vi "Save Profi map Power.vi"(7 "Write":bool, 8 "error in":errorcluster, 10 "configuration file path":path, 11 "Power Meters":cluster{"Select Item 3":T2, "Combo Box 2":T4}[](array[cluster])) -> (0 "error out":errorcluster, 3 "Array":cluster{"Sensor":T1, "Profi":T2}[](array[cluster]))   [LabVIEW 2025]
uses:
  <vilib>/Utility/config.llb/NI_LVConfig.lvlib
  controls/Tempratures.ctl
  controls/Profi address.ctl
  <vilib>/Utility/config.llb/Read Key (String).vi
  <vilib>/Utility/config.llb/Write Key (String).vi
  controls/Power Meters.ctl
panel:
  in  "Pressure":T3(array[cluster])
  in  "Tempratures":cluster{"Sensor":T1, "Profi":T2}[][](array[cluster])
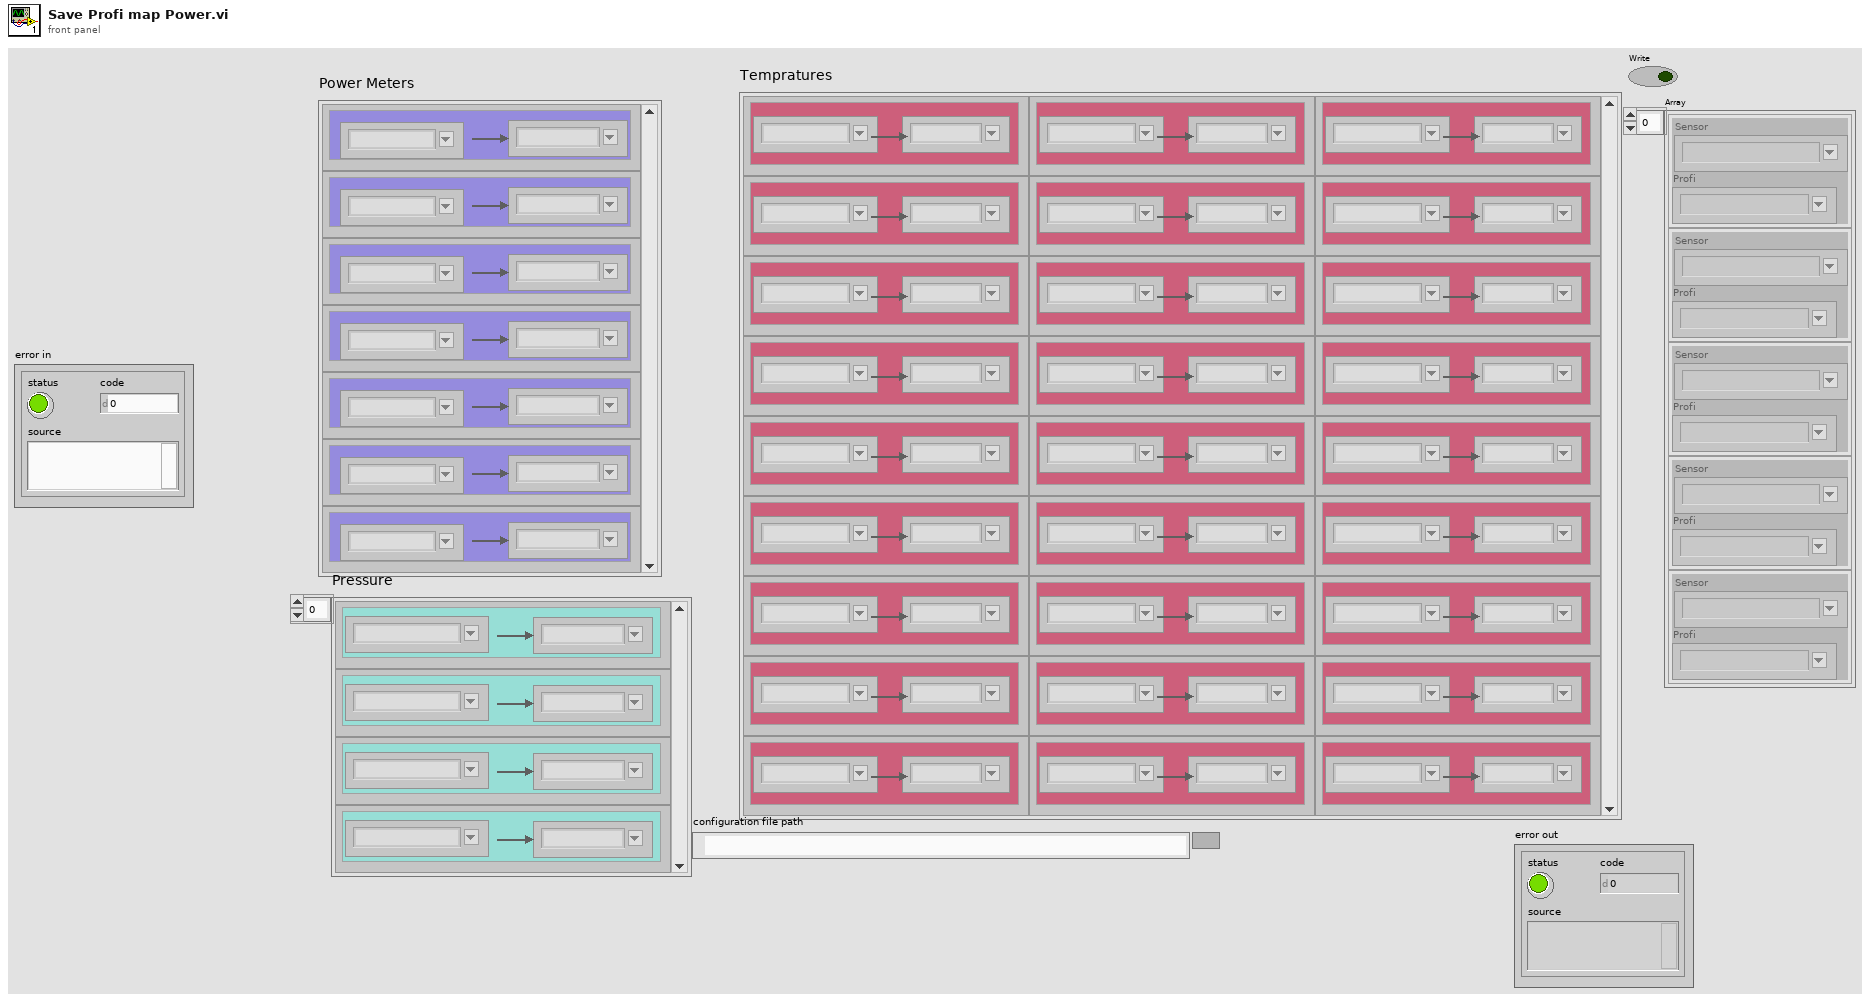
[diagram p1: front panel]
types:
  T1 = typedef "Tempratures.ctl" = string
  T2 = typedef "Profi address.ctl" = string
  T3 = cluster{"Select Item 3":T2, "Combo Box 2":string}[]
  T4 = typedef "Power Meters.ctl" = string
  T5 = typedef "NI_LVConfig.lvlib/Config Data RefNum.ctl" = refnum<k1>
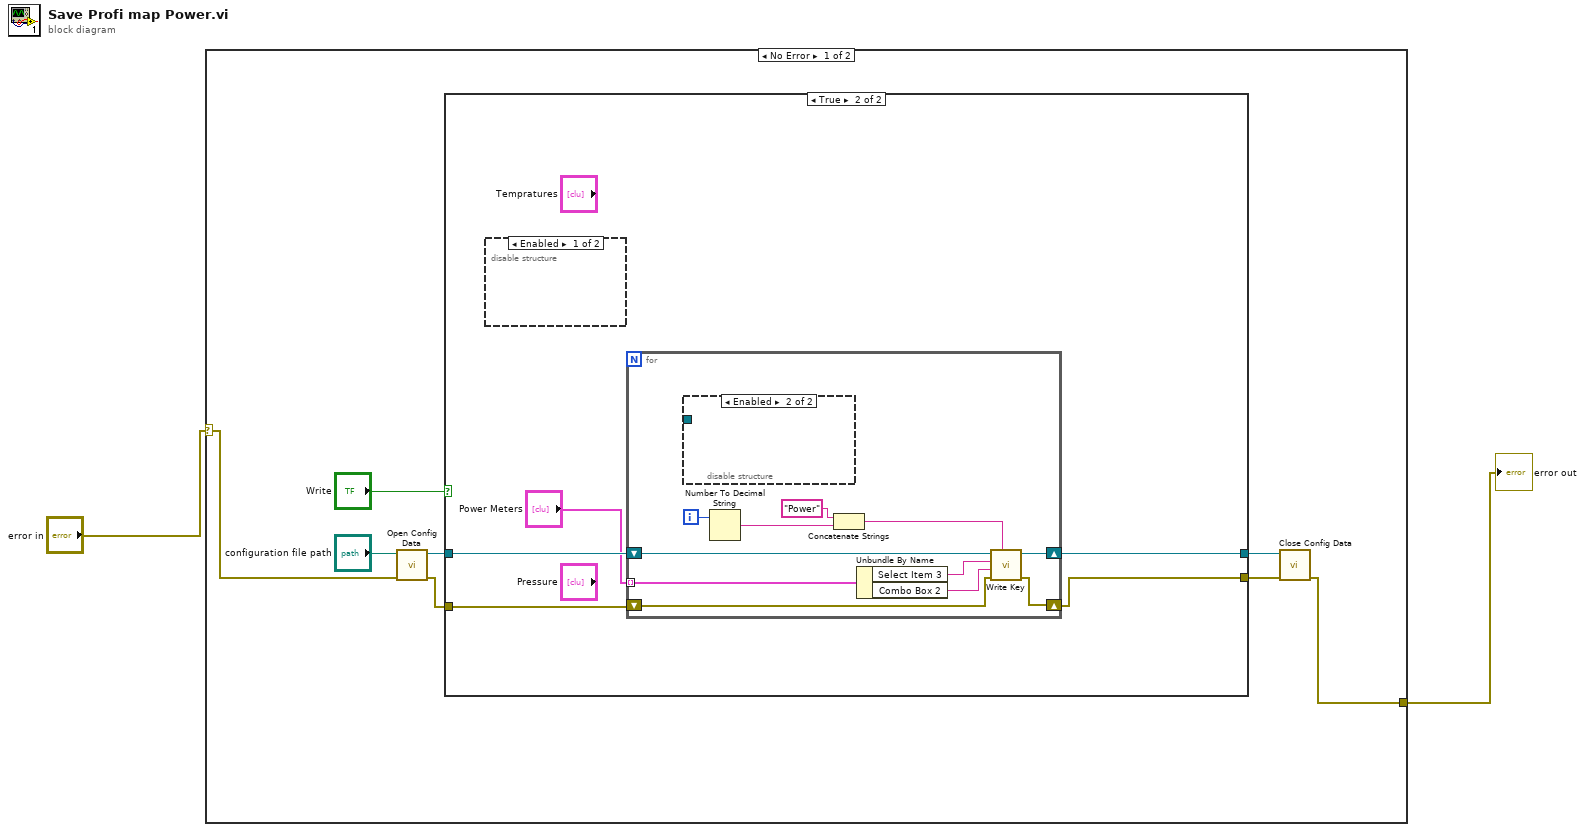
[diagram p0: block diagram]
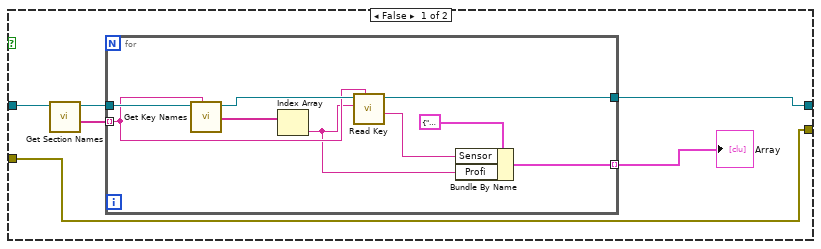
[diagram p2: hidden frame]
diagram:
  n1 = case shown="No Error" "error in" {
    selector: "error in" -> [w6 w43]
    tunnel: [w3 w43] -> w1
    frame No Error {
      n2 = call <vilib>:"Open Config Data.vi"("error in (no error)"=w6, "configuration file path"="configuration file path") -> ("error out"=w5:errorcluster, "refnum"=w10:T5)  [unwired: 7 in, 1 out]
      n3 = case shown="True" "Write" {
        tunnel: w10 -> [w15 w30]
        tunnel: [w16 w29] -> w7
        tunnel: w5 -> [w12 w27]
        tunnel: [w12 w26] -> w4
        frame False {
          n4 = call <vilib>:"Get Section Names.vi"("refnum"=w15) -> ("section names"=w14:string[], "refnum out"=w13:T5)  [unwired: 8 in, 1 out]
          n5 = for {
            tunnel: [w25] -> w16
            tunnel: w14 -> [w20] mode=indexing
            tunnel: w13 -> [w23]
            tunnel: [w22] -> w11 mode=indexing
            n6 = call <vilib>:"Get Key Names.vi"("section"=w20, "refnum"=w23) -> ("key names"=w19:string[], "refnum out"=w24:T5)  [unwired: 6 in, 2 out]
            n7 = Index Array(array=w19) -> (element=w17:string)  [unwired: 1 in]
            n8 = call-poly <vilib>:"Read Key.vi"("section"=w20, "key"=w17, "refnum"=w24) -> ("value"=w18:string, "refnum out"=w25:T5)  [unwired: 5 in, 2 out]
            n9 = Bundle By Name(cluster=cluster{"Sensor":T1, "Profi":T2} {"Sensor"="", "Profi"=""} ("Cluster 6"), "Sensor"=w18, "Profi"=w17) -> (w22:cluster{"Sensor":T1, "Profi":T2})
          }
          "Array" <- w11
        }
        frame True {
          n10 = disable-structure shown="Enabled" {
            frame Enabled {
            }
            frame Disabled {
            }
          }
          n11 = for {
            tunnel: "Power Meters" -> [w41] mode=indexing
            shift-right: [w39] -> w29
            shift-left: w30 -> [w40]
            shift-right: [w31] -> w26
            shift-left: w27 -> [w32]
            i -> [w33]
            n12 = disable-structure shown="Enabled" {
              disable-tunnel: _ -> [w42 _]
              frame Disabled {
              }
              frame Enabled {
              }
            }
            n13 = Number To Decimal String(number=w33) -> (decimal integer string=w35:string)  [unwired: 1 in]
            n14 = Concatenate Strings("Power", w35) -> (w34:string)
            n15 = Unbundle By Name(w41) -> ("Select Item 3"=w38:T2, "Combo Box 2"=w37:T4)
            n16 = call-poly <vilib>:"Write Key.vi"("section"=w34, "error in (no error)"=w32, "value"=w37, "key"=w38, "refnum"=w40) -> ("error out"=w31:errorcluster, "refnum out"=w39:T5)  [unwired: 4 in, 1 out]
          }
        }
      }
      n17 = call <vilib>:"Close Config Data.vi"("error in (no error)"=w4, "refnum"=w7) -> ("error out"=w3:errorcluster)  [unwired: 8 in, 1 out]
    }
    frame Error {
    }
  }
  "error out" <- w1
